vi "VM - 1D Array of CDB.vi"(6 "global? (F)":bool, 7 "VC Handle":T3=-1, 8 "error in":errorcluster, 9 "cmd":T2(ring)=enum."get value", 10 "value in":cdb[](array[numeric]), 11 "name_spec":string) -> (0 "error out":errorcluster, 1 "err code":T1 items=["No error", "Invalid variable type", "Variable not found", "Variable already exists", "Invalid context handle", "Input error", "Invalid data format", "No history attached", "History already attached", "Invalid history parameters", "Wrong variable name", "Wrong alias name", "Non-unique alias", "Alias not found", "No alias associated", "Alias already associated", "Wrong context name", "Non-unique context name", "Context name not found", "Invalid parameter", "Generic error", "Memory Full", "Unrecognized LV error", "Unknown error code"], 2 "value out":cdb[](array[numeric]), 3 "dup name_spec":string, 4 "global out":bool, 5 "dup VC Handle":T3=-1)   [LabVIEW 2021]
doc: "This VI manages variables of the <b>1D Array of CDB</b> data type. Refer to the VI help for more details.\n\n<b>VC Handle</b> specifies the handle of the variable context. This input is ignored if the <b>name_spec</b> control refers to a variable by an alias during 'get value', 'set value', and 'destroy' actions or if the action is 'create' and <b>global?</b> is TRUE.\n\n<b>name_spec</b> is the name specifier of the desired variable. Usually, it is merely a variable name; however, its generic format is '[name][=alias]', where either 'name' or '=alias' can be omitted but not both.\n\n<b>cmd</b> control specifies the action to be performed on the variable. Possible actions are 'create', 'destroy', 'get value', and 'set value'.\n\n<b>value in</b> control specifies the value to be written to the variable; it is only used during 'set value' or 'create' actions. <b>value out</b> indicator returns the value that has been read from the variable.\n\n<b>global?</b> control, if TRUE, enables access to global variables. For 'create' and 'destroy' actions, it causes the VI to ignore <b>VC Handle</b> and operate on a global variable. For 'get value' and 'set value' actions, it allows the VI to operate on a global variable if the specified variable name is not found in the context specified by <b>VC Handle</b>.\n\n<b>global out</b> indicator returns TRUE if an action has been performed on a global variable.\n\n<b>err code</b> indicator returns a VarMan Engine error code.\n\n::: CalcExpress Toolkit :::\nCopyright (c) 2000-2026 Konstantin Shifershteyn. All rights reserved."
uses:
  cetypes.llb/VarMan Variable Context Handle.ctl
  cetypes.llb/VarMan Error Code.ctl
  cersrc/celveng32.dll
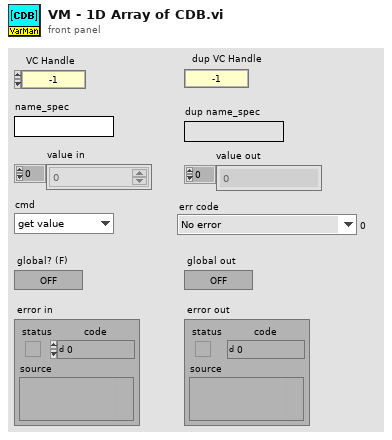
[diagram p1: front panel]
types:
  T1 = typedef "VarMan Error Code.ctl" = u16
  T2 = enum16{"create", "destroy", "set value", "get value"}
  T3 = typedef "VarMan Variable Context Handle.ctl" = i32
  T4 = enum32{"String", "DBL Number", "identifier", "1D Array of DBL", "2D Array of DBL", "CDB Number", "1D Array of CDB", "2D Array of CDB", "1D Array of String", "2D Array of String", "Unknown data type"}
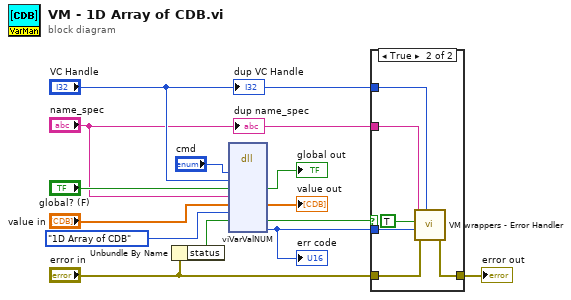
[diagram p0: block diagram]
diagram:
  n1 = Unbundle By Name("error in") -> ("status"=w10:bool)
  n2 = dll-call lib="C:/LV Projects/CalcExpress 40 LV2021/vi.lib/addons/CalcExpress/cersrc/celveng*.dll" fn="viVarValNUM"("cmd"="cmd", "vch"="VC Handle", "gbl"="global? (F)", "name"="name_spec", "val"="value in", "type"=T4."1D Array of CDB" ("data type"), "errf"=w10) -> ("gbl"=→"global out":bool, "val"=→"value out":cdb[], "errf"=w4:bool, "err code"=w11:T1)  [unwired: 9 in, 2 out]
  "err code" <- w11
  n3 = case shown="True" w4 {
    tunnel: [w14 w20] -> w13
    tunnel: "error in" -> [w14 w19]
    tunnel: w11 -> [_ w18]
    tunnel: "VC Handle" -> [_ w16]
    tunnel: "name_spec" -> [_ w15]
    frame False {
    }
    frame True {
      n4 = call "VM wrappers - Error Handler.vi"("VC Handle"=w16, "error before"=w19, "VarMan error"=w18, "show name spec (F)"=TRUE, "name spec"=w15) -> ("error out"=w20:errorcluster)  [unwired: 5 in, 1 out]
    }
  }
  "error out" <- w13
  "dup VC Handle" <- "VC Handle"
  "dup name_spec" <- "name_spec"
